vi "Get Class List from Folder.vi"(8 "error in (no error)":errorcluster, 11 "Folder Path":path) -> (0 "error out":errorcluster, 3 "Class List[]":path[](array[path]))   [LabVIEW 2016, in "SLL Class.lvlib"]
doc: "Get list of classes present in a given folder, including classes that are present inside LabVIEW Packed Project Library (PPLs)"
uses:
  SLL Class.lvlib
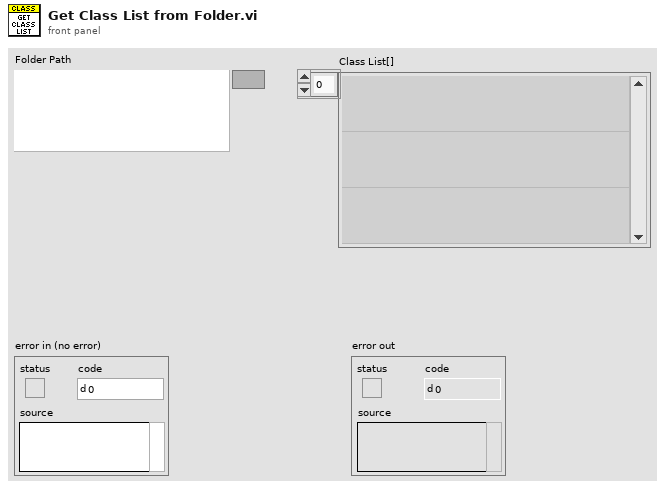
[diagram p1: front panel]
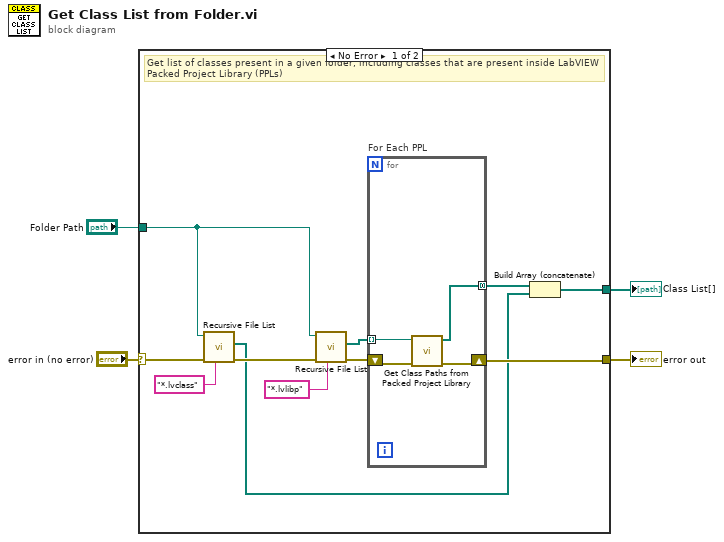
[diagram p0: block diagram]
diagram:
  n1 = case shown="No Error" "error in (no error)" {
    selector: "error in (no error)" -> [w15 w20]
    tunnel: [w8 w20] -> w3
    tunnel: "Folder Path" -> [w12 _]
    tunnel: [w5 _] -> w1
    frame No Error {
      # "Get list of classes present in a given folder, including classes that are present inside LabVIEW Packed Project Library (PPLs)"
      n2 = call <vilib>:"Recursive File List.vi"("pattern"="*.lvclass", "error in (no error)"=w15, "Folder Path"=w12) -> ("error out"=w13:errorcluster, "All Files in Dir"=w7:path[])  [unwired: 4 in, 3 out]
      n3 = call <vilib>:"Recursive File List.vi"("pattern"="*.lvlibp", "error in (no error)"=w13, "Folder Path"=w12) -> ("error out"=w10:errorcluster, "All Files in Dir"=w9:path[])  [unwired: 4 in, 3 out]
      n4 = for "For Each PPL" {
        tunnel: w9 -> [w18] mode=indexing
        shift-right: [w17] -> w8
        shift-left: w10 -> [w19]
        tunnel: [w16] -> w6 mode=concatenating
        n5 = call "Get Class Paths from Packed Project Library.vi"("error in (no error)"=w19, "Packed Library Path"=w18) -> ("error out"=w17:errorcluster, "Class List[]"=w16:path[])  [unwired: 8 in]
      }
      n6 = Build Array (concatenate)(w6, w7) -> (w5:path[])
    }
    frame Error {
    }
  }
  "error out" <- w3
  "Class List[]" <- w1
